vi "Generate GraphViz Mapping File.vi"(7 "supported colors":string[](array[string])=["dodgerblue", "cadetblue1", "darkgoldenrod1", "gainsboro"], 8 "Show Unmapped Channels?":bool=TRUE, 9 "Show Tag Labels?":bool=TRUE, 10 "Modules Configurations":refnum<class "TBM module configuration.lvclass">[](array[class]), 11 "engine configuration in":refnum<class "engine configuration.lvclass">) -> (3 "output to graphviz":string)   [LabVIEW 2014, in "GraphViz Mapping Visualizer.lvlib"]
uses:
  GraphViz Mapping Visualizer.lvlib
  <vilib>/NI/Tag Bus Module Framework/module configuration/TBM module configuration.lvclass
  <vilib>/NI/Module Execution Interface/Engine Configuration/engine configuration.lvclass
  Channel to Port Pair.ctl
  <vilib>/NI/Tag Bus/tag/Data Type.ctl
  <vilib>/NI/Tag Bus/tag/tag descriptor.lvclass/tag descriptor.ctl
  <vilib>/NI/Tag Bus Module Framework/channel/channel classification.ctl
  <vilib>/NI/Tag Bus/tag/read tag name.vi
  <vilib>/NI/Tag Bus/tag/read data type.vi
  <vilib>/NI/Tag Bus Module Framework/channel/TBM channel.lvclass
  Configuration Editor/Classes/Engine Mappings/Engine Mappings.lvclass
  <vilib>/NI/Tag Bus/tag/tag descriptor.lvclass
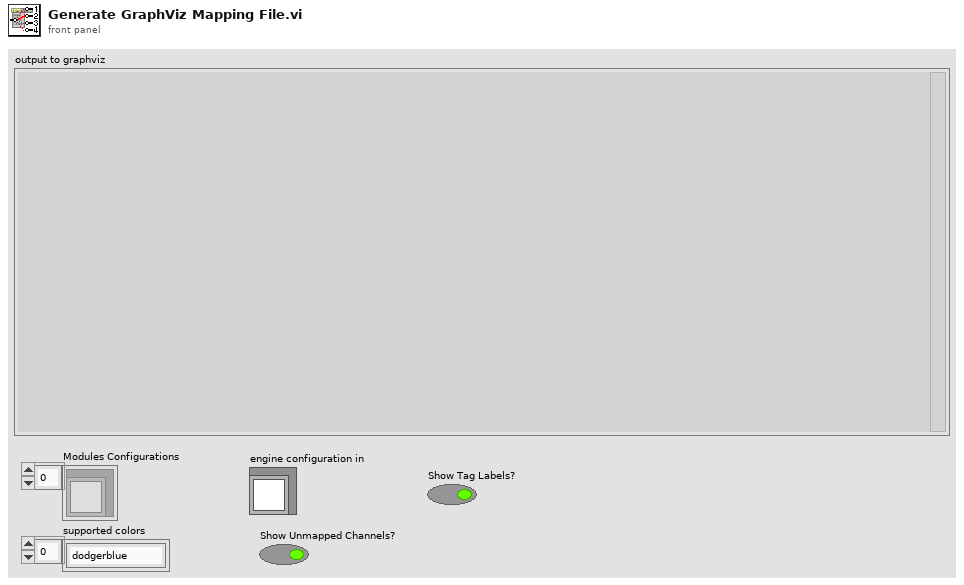
[diagram p1: front panel]
types:
  T1 = typedef "GraphViz Mapping Visualizer.lvlib/Channel to Port Pair.ctl" = cluster{"Channel Name":string, "Node:Port":string}
  T2 = typedef "PL Framework Configuration Tool.lvlib/Engine Mappings.lvclass/module information.ctl" = cluster{"display name":string, "instance id":string, "channels":refnum<class "TBM channel.lvclass">[]}
  T3 = typedef "engine configuration.lvclass/Tag Info.ctl" = cluster{"Tag":refnum<class "tag descriptor.lvclass">, "Writer Module":string, "Writer Channel":string, "Readers":cluster{"module":string, "channel":string}[], "Owning ID":string}
  T4 = typedef "tag bus.lvlib/tag descriptor.lvclass/Data Type.ctl" = enum16{"Double", "Single", "I64", "I32", "I16", "I8", "U64", "U32", "U16", "U8", "Boolean", "String", "Array of Double", "Array of Single", "Array of I64", "Array of I32", "Array of I16", "Array of I8", "Array of U64", "Array of U32", "Array of U16", "Array of U8", "Array of Boolean", "Array of String"}
  T5 = cluster{"name":string, "data type":T4, "writer":string, "readers":string[]}
  T6 = typedef "TBM channel.lvclass/channel classification.ctl" = enum16{"input data", "output data", "processing parameter", "processing result"}
  T7 = cluster{"Instance ID":string, "name":string, "default value string":string, "index":i32}[]
  T8 = cluster{"display strings and indices":cluster{"Instance ID":string, "name":string, "default value string":string, "index":i32}[], "display strings and indices":cluster{"Instance ID":string, "name":string, "default value string":string, "index":i32}[]}
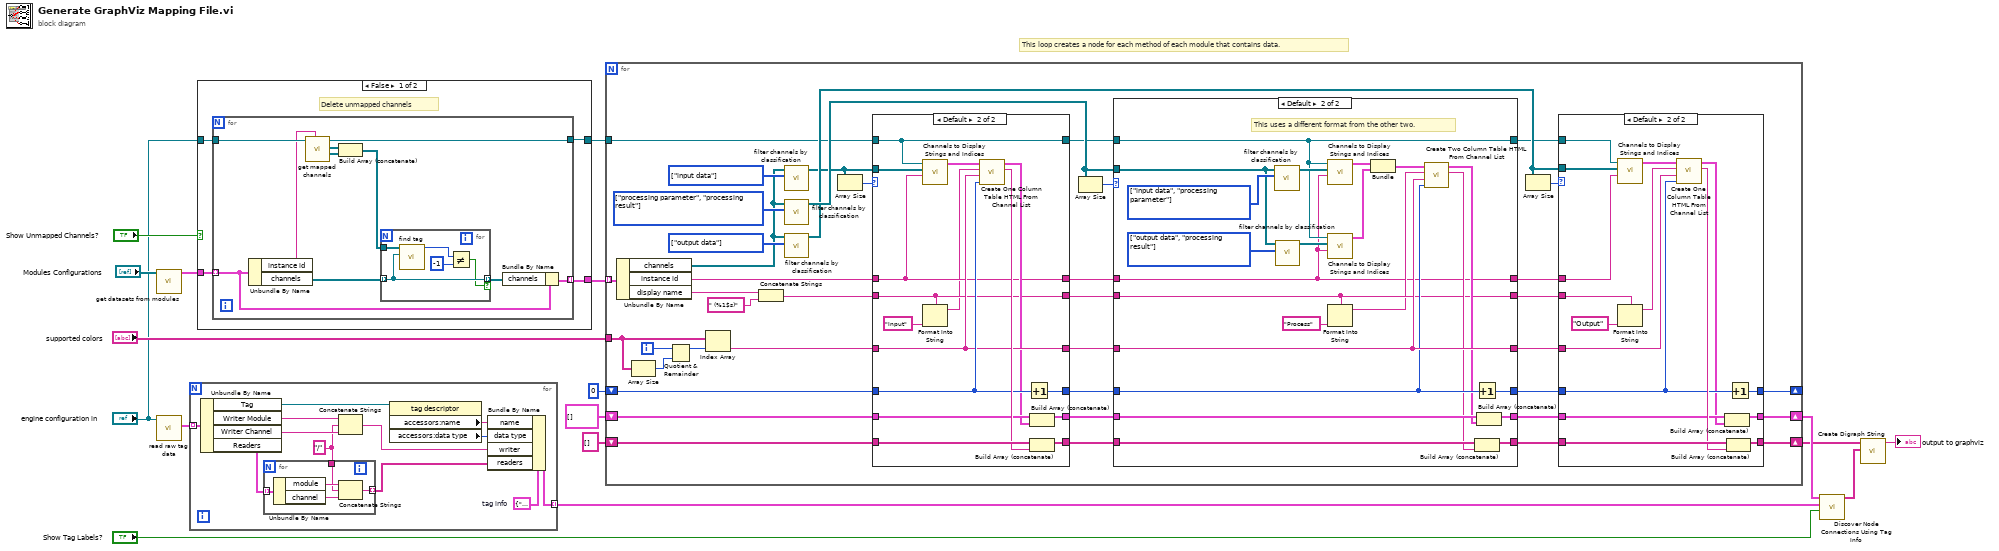
[diagram p0: block diagram]
diagram:
  # "This loop creates a node for each method of each module that contains data."
  n1 = call "get datasets from modules.vi"("Modules Configurations"="Modules Configurations") -> ("module datasets"=w11:T2[])  [unwired: 9 in, 1 out]
  n2 = call <vilib>:"read raw tag data.vi"("engine configuration in"="engine configuration in") -> ("raw tag data"=w6:T3[])  [unwired: 8 in, 2 out]
  n3 = for {
    tunnel: w6 -> [w25] mode=indexing
    tunnel: [w19] -> w4 mode=indexing
    w20 = T5 {"name"="", "data type"=enum."Double", "writer"="", "readers"=[]}  # tag info
    w18 = "/" ("string")
    n4 = Unbundle By Name(w25) -> ("Tag"=w26:refnum<class "tag descriptor.lvclass">, "Writer Module"=w28:string, "Writer Channel"=w29:string, "Readers"=w27:cluster{"module":string, "channel":string}[])
    n5 = for {
      tunnel: w27 -> [w34] mode=indexing
      tunnel: [w31] -> w21 mode=indexing
      tunnel: w18 -> [w30]
      n6 = Unbundle By Name(w34) -> ("module"=w33:string, "channel"=w32:string)
      n7 = Concatenate Strings(w33, w30, w32) -> (w31:string)
    }
    n8 = Concatenate Strings(w28, w18, w29) -> (w22:string)
    n9 = property class="tag descriptor"(reference=w26) -> ("accessors:name"=w24:string, "accessors:data type"=w23:T4)  [unwired: 1 in, 2 out]
    n10 = Bundle By Name(cluster=w20, "name"=w24, "data type"=w23, "writer"=w22, "readers"=w21) -> (w19:T5)
  }
  n11 = case shown="False" "Show Unmapped Channels?" {
    tunnel: w11 -> [w38 w55]
    tunnel: [w35 w55] -> w10
    tunnel: "engine configuration in" -> [w37 w54]
    tunnel: [w36 w54] -> w9
    frame False {
      # "Delete unmapped channels"
      n12 = for {
        tunnel: w38 -> [w44] mode=indexing
        tunnel: w37 -> [w48]
        tunnel: [w47] -> w36
        tunnel: [w42] -> w35 mode=indexing
        n13 = Unbundle By Name(w44) -> ("instance id"=w46:string, "channels"=w45:refnum<class "TBM channel.lvclass">[])
        n14 = call-dynamic "get mapped channels.vi"("owner"=w46, "engine configuration in"=w48) -> ("write channels"=w40:refnum<class "TBM channel.lvclass">[], "read channels"=w41:refnum<class "TBM channel.lvclass">[], "engine configuration out"=w47:refnum<class "engine configuration.lvclass">)  [unwired: 5 in, 2 out]
        n15 = Build Array (concatenate)(w41, w40) -> (w39:refnum<class "TBM channel.lvclass">[])
        n16 = for {
          tunnel: w39 -> [w51]
          tunnel: w45 -> [w50] mode=indexing
          tunnel: [w50] -> w43 mode=indexing if=w49
          n17 = call <vilib>:"find tag.vi"("tag"=w50, "tags in"=w51) -> ("index"=w52:i32)  [unwired: 9 in]
          n18 = Not Equal?(x=w52, y=-1 ("x")) -> (x != y?=w49:bool)
        }
        n19 = Bundle By Name(cluster=w44, "channels"=w43) -> (w42:T2)
      }
    }
    frame True {
    }
  }
  n20 = for {
    tunnel: w10 -> [w96] mode=indexing
    shift-right: [w84] -> w2
    shift-left: string[] [] -> [w94]
    shift-right: [w83] -> _
    shift-left: 0 -> [w91]
    shift-right: [w80] -> w5
    shift-left: T1[] [] -> [w81]
    tunnel: "supported colors" -> [w75]
    tunnel: w9 -> [w62]
    i -> [w74]
    w65 = T6[] [enum."output data"] items=["input data", "output data", "processing parameter", "processing result"] ("allowed classifications")
    w67 = T6[] [enum."processing parameter", enum."processing result"] items=["input data", "output data", "processing parameter", "processing result"] ("allowed classifications")
    w68 = T6[] [enum."input data"] items=["input data", "output data", "processing parameter", "processing result"] ("allowed classifications")
    n21 = Unbundle By Name(w96) -> ("channels"=w64:refnum<class "TBM channel.lvclass">[], "instance id"=w82:string, "display name"=w57:string)
    n22 = Array Size(array=w75) -> (size(s)=w73:i32)
    n23 = Quotient & Remainder(x=w74, y=w73) -> (x-y*floor(x/y)=w72:i32)  [unwired: 1 out]
    n24 = Index Array(array=w75, index=w72) -> (element=w71:string)
    n25 = Concatenate Strings(w57, " (%1$s)" ("format string")) -> (w58:string)
    n26 = call <vilib>:"filter channels by classification.vi"("allowed classifications"=w68, "channels in"=w64) -> ("channels out"=w56:refnum<class "TBM channel.lvclass">[])  [unwired: 9 in]
    n27 = call <vilib>:"filter channels by classification.vi"("allowed classifications"=w67, "channels in"=w64) -> ("channels out"=w66:refnum<class "TBM channel.lvclass">[])  [unwired: 9 in]
    n28 = call <vilib>:"filter channels by classification.vi"("allowed classifications"=w65, "channels in"=w64) -> ("channels out"=w63:refnum<class "TBM channel.lvclass">[])  [unwired: 9 in]
    n29 = Array Size(array=w56) -> (size(s)=w95:i32)
    n30 = case shown="Default" w95 {
      tunnel: w56 -> [_ w157]
      tunnel: [w151 w167] -> w93
      tunnel: w94 -> [w151 w166]
      tunnel: w58 -> [w149 w154]
      tunnel: w91 -> [w150 w162]
      tunnel: [w150 w165] -> w89
      tunnel: [w149 w154] -> w90
      tunnel: w82 -> [w147 w156]
      tunnel: w81 -> [w148 w163]
      tunnel: [w148 w161] -> w78
      tunnel: [w147 w156] -> w77
      tunnel: w71 -> [w146 w160]
      tunnel: [w146 w160] -> w70
      tunnel: w62 -> [w145 w158]
      tunnel: [w145 w158] -> w61
      frame 0 {
        # "don't create a node if there are no channels of that type"
      }
      frame Default {
        n31 = call "Channels to Display Strings and Indices.vi"("Instance ID"=w156, "Channels"=w157, "engine configuration in"=w158) -> ("display strings and indices"=w155:T7)  [unwired: 8 in]
        n32 = Format Into String(format string=w154, "Input" ("string")) -> (resulting string=w152:string)  [unwired: 2 in, 1 out]
        n33 = call "Create One Column Table HTML From Channel List.vi"("Node#"=w162, "Color"=w160, "Title"=w152, "display strings and indices"=w155) -> ("Table HTML"=w164:string, "Channel and Node Pairs"=w159:T1[])  [unwired: 6 in]
        n34 = Increment(x=w162) -> (x+1=w165:i32)
        n35 = Build Array (concatenate)(w163, w159) -> (w161:T1[])
        n36 = Build Array (concatenate)(w166, w164) -> (w167:string[])
      }
    }
    n37 = Array Size(array=w66) -> (size(s)=w92:i32)
    n38 = case shown="Default" w92 {
      tunnel: w66 -> [_ w125]
      tunnel: [w122 w144] -> w87
      tunnel: w93 -> [w122 w143]
      tunnel: w90 -> [w120 w135]
      tunnel: w89 -> [w121 w138]
      tunnel: [w121 w142] -> w88
      tunnel: [w120 w135] -> w86
      tunnel: [w119 w141] -> w79
      tunnel: w78 -> [w119 w140]
      tunnel: w77 -> [w118 w124]
      tunnel: [w118 w124] -> w76
      tunnel: w70 -> [w117 w139]
      tunnel: [w117 w139] -> w69
      tunnel: w61 -> [w116 w126]
      tunnel: [w116 w126] -> w60
      frame 0 {
        # "don't create a node if there are no channels of that type"
      }
      frame Default {
        w131 = T6[] [enum."output data", enum."processing result"] items=["input data", "output data", "processing parameter", "processing result"] ("allowed classifications")
        w132 = T6[] [enum."input data", enum."processing parameter"] items=["input data", "output data", "processing parameter", "processing result"] ("allowed classifications")
        # "This uses a different format from the other two."
        n39 = call <vilib>:"filter channels by classification.vi"("allowed classifications"=w132, "channels in"=w125) -> ("channels out"=w130:refnum<class "TBM channel.lvclass">[])  [unwired: 9 in]
        n40 = call <vilib>:"filter channels by classification.vi"("allowed classifications"=w131, "channels in"=w125) -> ("channels out"=w129:refnum<class "TBM channel.lvclass">[])  [unwired: 9 in]
        n41 = call "Channels to Display Strings and Indices.vi"("Instance ID"=w124, "Channels"=w130, "engine configuration in"=w126) -> ("display strings and indices"=w128:T7)  [unwired: 8 in]
        n42 = call "Channels to Display Strings and Indices.vi"("Instance ID"=w124, "Channels"=w129, "engine configuration in"=w126) -> ("display strings and indices"=w127:T7)  [unwired: 8 in]
        n43 = Format Into String(format string=w135, "Process" ("string")) -> (resulting string=w133:string)  [unwired: 2 in, 1 out]
        n44 = Bundle("display strings and indices"=w128, "display strings and indices"=w127) -> (w123:T8)  [unwired: 1 in]
        n45 = call "Create Two Column Table HTML From Channel List.vi"("Node#"=w138, "Color"=w139, "Title"=w133, "process display strings and indices"=w123) -> ("Table HTML"=w137:string, "Channel and Node Pairs"=w136:T1[])  [unwired: 6 in]
        n46 = Increment(x=w138) -> (x+1=w142:i32)
        n47 = Build Array (concatenate)(w143, w137) -> (w144:string[])
        n48 = Build Array (concatenate)(w140, w136) -> (w141:T1[])
      }
    }
    n49 = Array Size(array=w63) -> (size(s)=w85:i32)
    n50 = case shown="Default" w85 {
      tunnel: w63 -> [_ w105]
      tunnel: [w99 w115] -> w84
      tunnel: w87 -> [w99 w114]
      tunnel: w86 -> [_ w102]
      tunnel: w88 -> [w98 w109]
      tunnel: [w98 w112] -> w83
      tunnel: [w97 w111] -> w80
      tunnel: w79 -> [w97 w110]
      tunnel: w76 -> [_ w103]
      tunnel: w69 -> [_ w108]
      tunnel: w60 -> [_ w106]
      frame 0 {
        # "don't create a node if there are no channels of that type"
      }
      frame Default {
        n51 = call "Channels to Display Strings and Indices.vi"("Instance ID"=w103, "Channels"=w105, "engine configuration in"=w106) -> ("display strings and indices"=w104:T7)  [unwired: 8 in]
        n52 = Format Into String(format string=w102, "Output" ("string")) -> (resulting string=w101:string)  [unwired: 2 in, 1 out]
        n53 = call "Create One Column Table HTML From Channel List.vi"("Node#"=w109, "Color"=w108, "Title"=w101, "display strings and indices"=w104) -> ("Table HTML"=w113:string, "Channel and Node Pairs"=w107:T1[])  [unwired: 6 in]
        n54 = Build Array (concatenate)(w110, w107) -> (w111:T1[])
        n55 = Build Array (concatenate)(w114, w113) -> (w115:string[])
        n56 = Increment(x=w109) -> (x+1=w112:i32)
      }
    }
  }
  n57 = call "Discover Node Connections Using Tag Info.vi"("Show Tag Labels?"="Show Tag Labels?", "tag info"=w4, "channel and node pairs"=w5) -> ("node connections"=w1:string[][])  [unwired: 8 in]
  n58 = call "Create Digraph String.vi"("node connections"=w1, "tables html"=w2) -> ("digraph output"=→"output to graphviz":string)  [unwired: 9 in]
